vi "PicoScope4000Settings.vi"(0 "handle in":i16, 3 "Unit Info":T1, 5 "error in":errorcluster, 6 "Channel A Settings":T3 {"Coupling" items=["AC", "DC", "IEPE"]; "Bandwidth Limit" items=["Off", "200kHz"]; "Range" items=["10 mV", "20 mV", "50 mV", "100 mV", "200 mV", "500 mV", "1 V", "2 V", "5 V", "10 V", "20 V", "50 V ", "100 V"]}, 7 "Trigger Settings":T4 {"Trigger Direction" items=["Rising", "Falling"]}, 8 "Channel B Settings":T3 {"Coupling" items=["AC", "DC", "IEPE"]; "Bandwidth Limit" items=["Off", "200kHz"]; "Range" items=["10 mV", "20 mV", "50 mV", "100 mV", "200 mV", "500 mV", "1 V", "2 V", "5 V", "10 V", "20 V", "50 V ", "100 V"]}, 10 "Channel C Settings":T2 {"Range" items=["10 mV", "20 mV", "50 mV", "100 mV", "200 mV", "500 mV", "1 V", "2 V", "5 V", "10 V", "20 V", "50 V ", "100 V"]; "Coupling" items=["AC", "DC"]}, 12 "Channel D Settings":T2 {"Range" items=["10 mV", "20 mV", "50 mV", "100 mV", "200 mV", "500 mV", "1 V", "2 V", "5 V", "10 V", "20 V", "50 V ", "100 V"]; "Coupling" items=["AC", "DC"]}, 13 "PicoScope 4262 Ext. Trigger Range":u32(ring) items=["500 mV", "5 V"]) -> (11 "Enabled array":i16[](array[numeric]), 14 "handle out":i16, 19 "error out":errorcluster)   [LabVIEW 2009]
doc: "This VI is used to set up the oscilloscope. The inputs are clusters for setting channel and simple trigger settings. Advanced triggers can be set up using PicoScope4000AdvancedTriggerSettings.vi"
uses:
  ps4000.dll
  PicoScope4000AnalogChannelSettings.ctl
  PicoScope4000AnalogChannelSettingsIEPE.ctl
panel:
  in  "Max ADC value":i16
  # "Note Bandwith Limit not avaiable on all models"
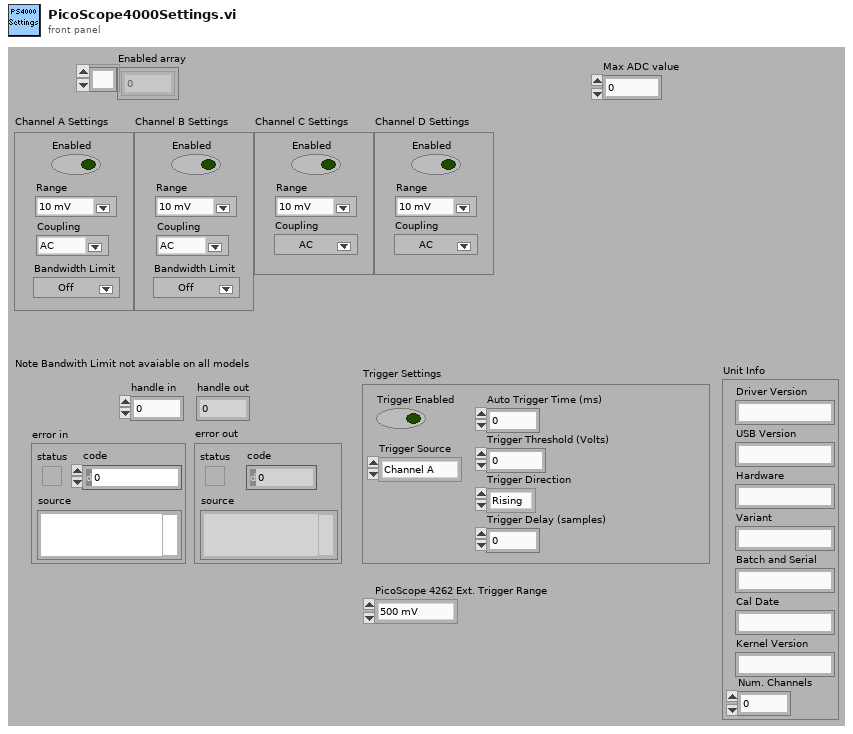
[diagram p1: front panel]
types:
  T1 = cluster{"Driver Version":string, "USB Version":string, "Hardware":string, "Variant":string, "Batch and Serial":string, "Cal Date":string, "Kernel Version":string, "Num. Channels":i16}
  T2 = typedef "PicoScope4000AnalogChannelSettings.ctl" = cluster{"Enabled":bool, "Coupling":i16, "Range":u16}
  T3 = typedef "PicoScope4000AnalogChannelSettingsIEPE.ctl" = cluster{"Enabled":bool, "Range":u16, "Bandwidth Limit":i16, "Coupling":u16}
  T4 = cluster{"Trigger Enabled":bool, "Trigger Source":enum16{"Channel A", "Channel B", "Channel C", "Channel D", "Channel E", "Channel F", "Channel G", "Channel H"}, "Trigger Threshold (Volts)":dbl, "Trigger Direction":u16, "Trigger Delay (samples)":u32, "Auto Trigger Time (ms)":i16}
  T5 = enum16{"Channel A", "Channel B", "Channel C", "Channel D", "Channel E", "Channel F", "Channel G", "Channel H"}
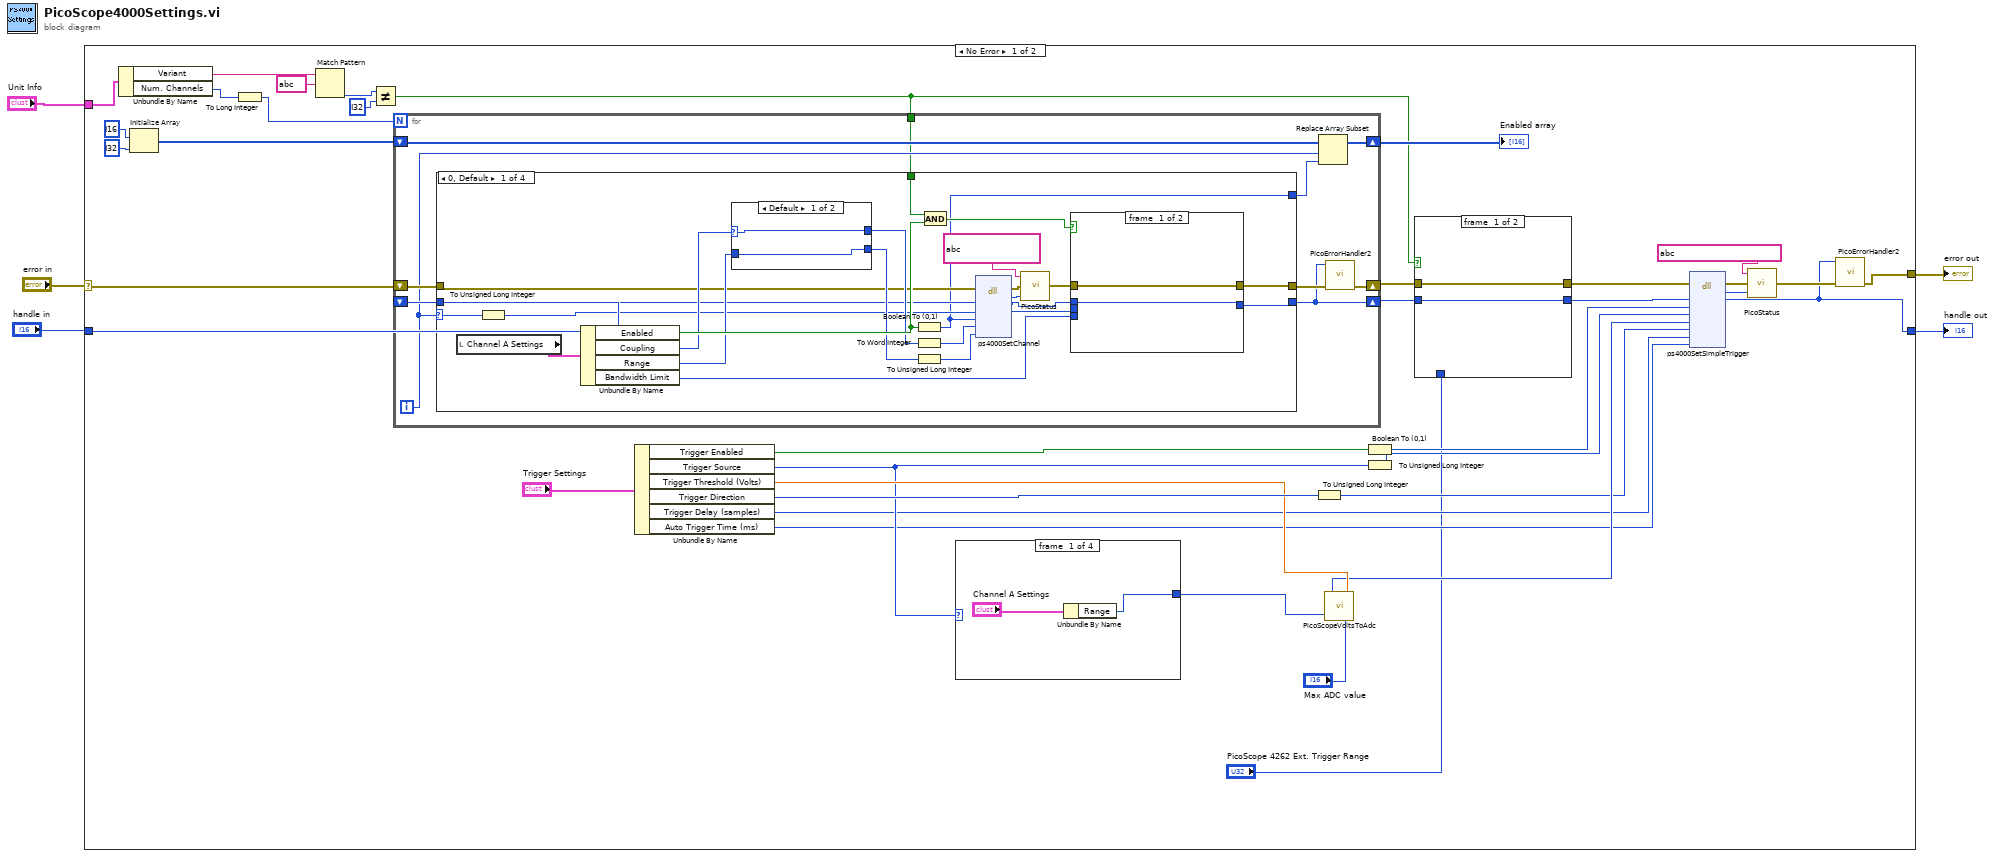
[diagram p0: block diagram]
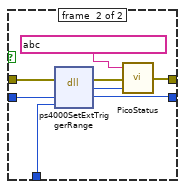
[diagram p2: hidden frame]
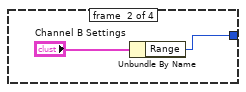
[diagram p3: hidden frame]
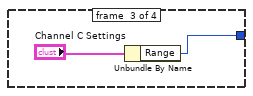
[diagram p4: hidden frame]
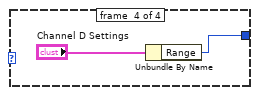
[diagram p5: hidden frame]
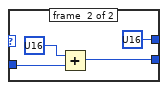
[diagram p6: hidden frame]
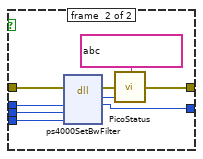
[diagram p7: hidden frame]
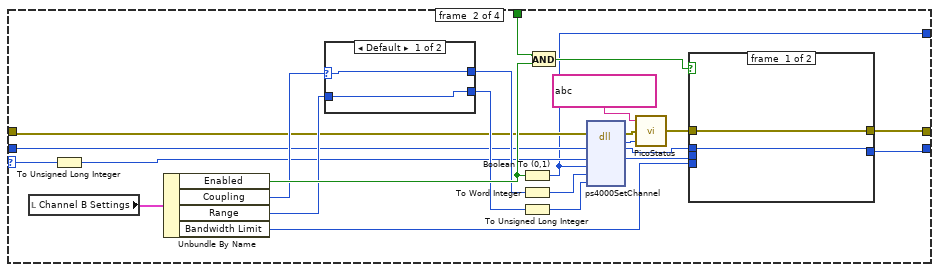
[diagram p8: hidden frame]
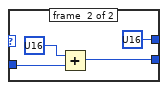
[diagram p9: hidden frame]
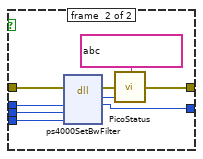
[diagram p10: hidden frame]
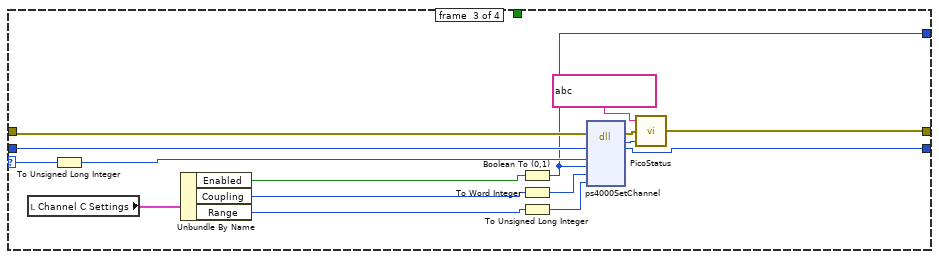
[diagram p11: hidden frame]
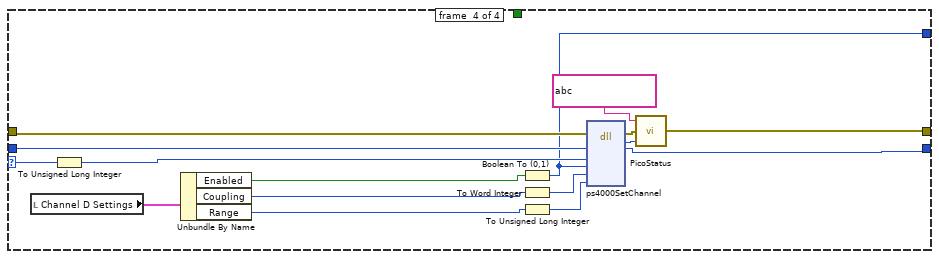
[diagram p12: hidden frame]
diagram:
  n1 = case shown="No Error" "error in" {
    selector: "error in" -> [w39 w187]
    tunnel: "handle in" -> [w40 w186]
    tunnel: [w6 w186] -> w3
    tunnel: [w7 w187] -> w2
    tunnel: "Unit Info" -> [w34 _]
    frame #0 {
      n2 = Unbundle By Name(w34) -> ("Variant"=w27:string, "Num. Channels"=w28:i16)
      n3 = Initialize Array(i16 ? ("element"), i32 ? ("dimension size")) -> (w36:i16[])
      n4 = To Long Integer(number=w28) -> (32bit integer=w33:i32)
      n5 = Match Pattern(string=w27, regular expression=string ?) -> (offset past match=w25:i32)  [unwired: 1 in, 3 out]
      n6 = Not Equal?(x=w25, y=i32 ?) -> (x != y?=w12:bool)
      n7 = for {
        N: w33 -> [_]
        shift-right: [w64] -> w11
        shift-left: w39 -> [w70]
        shift-right: [w63] -> w10
        shift-left: w40 -> [w71]
        shift-right: [w66] -> w35
        shift-left: w36 -> [w67]
        tunnel: w12 -> [w62]
        i -> [w69]
        n8 = case shown="0, Default" w69 {
          selector: w69 -> [w93 w135 w168 w184]
          tunnel: w71 -> [w78 w120 w163 w179]
          tunnel: [w91 w133 w156 w171] -> w65
          tunnel: w70 -> [w79 w121 w164 w180]
          tunnel: [w90 w132 w155 w172] -> w63
          tunnel: [w76 w118 w161 w177] -> w68
          tunnel: w62 -> [w88 w130 _ _]
          frame #0 {
            n9 = local read "Channel A Settings"() -> (w94:T3)
            n10 = To Unsigned Long Integer(number=w93) -> (unsigned 32bit integer=w77:u32)
            n11 = Unbundle By Name(w94) -> ("Enabled"=w87:bool, "Coupling"=w85:u16, "Range"=w82:u16, "Bandwidth Limit"=w86:i16)
            n12 = case shown="Default" w85 {
              selector: w85 -> [w96 _]
              tunnel: w82 -> [w97 w100]
              tunnel: [w97 w101] -> w83
              tunnel: [w96 u16 ? ("Coupling")] -> w84
              frame #0 {
              }
              frame #1 {
                n13 = Add(x=u16 ? ("y"), y=w100) -> (x+y=w101:u16)
              }
            }
            n14 = Boolean To (0,1)(Boolean=w87) -> (0, 1=w76:i16)
            n15 = To Word Integer(number=w84) -> (16bit integer=w75:i16)
            n16 = To Unsigned Long Integer(number=w83) -> (unsigned 32bit integer=w74:u32)
            n17 = And(x=w88, y=w87) -> (x .and. y?=w89:bool)
            n18 = dll-call lib="ps4000.dll" fn="ps4000SetChannel" ("ps3000.dll:_ps3000_open_unit@0")(error in=w79, "handle"=w78, "channel"=w77, "enabled"=w76, "dc"=w75, "range"=w74) -> (error out=w81:errorcluster, "PICO_STATUS"=w80:u32, "handle"=w73:i16, "channel"=w72:u32)  [unwired: 5 in, 1 out]
            n19 = call "PicoStatus.vi"("PICO STATUS"=w80, "error in"=w81, "source"=string ?) -> ("error out"=w92:errorcluster)
            n20 = case shown="True" w89 {
              tunnel: w92 -> [w103 w110]
              tunnel: w73 -> [w102 w109]
              tunnel: [w103 w108] -> w91
              tunnel: [w102 w107] -> w90
              tunnel: w72 -> [_ w105]
              tunnel: w86 -> [_ w104]
              frame #0 {
              }
              frame #1 {
                n21 = dll-call lib="ps4000.dll" fn="ps4000SetBwFilter" ("ps3000.dll:_ps3000_open_unit@0")(error in=w110, "handle"=w109, "channel"=w105, "enable"=w104) -> (error out=w112:errorcluster, "PICO_STATUS"=w106:u32, "handle"=w107:i16)  [unwired: 4 in, 1 out]
                n22 = call "PicoStatus.vi"("PICO STATUS"=w106, "error in"=w112, "source"=string ?) -> ("error out"=w108:errorcluster)
              }
            }
          }
          frame #1 {
            n23 = local read "Channel B Settings"() -> (w113:T3)
            n24 = To Unsigned Long Integer(number=w135) -> (unsigned 32bit integer=w119:u32)
            n25 = Unbundle By Name(w113) -> ("Enabled"=w129:bool, "Coupling"=w127:u16, "Range"=w124:u16, "Bandwidth Limit"=w128:i16)
            n26 = case shown="Default" w127 {
              selector: w127 -> [w137 _]
              tunnel: w124 -> [w138 w141]
              tunnel: [w138 w142] -> w125
              tunnel: [w137 u16 ? ("Coupling")] -> w126
              frame #0 {
              }
              frame #1 {
                n27 = Add(x=u16 ? ("y"), y=w141) -> (x+y=w142:u16)
              }
            }
            n28 = Boolean To (0,1)(Boolean=w129) -> (0, 1=w118:i16)
            n29 = To Word Integer(number=w126) -> (16bit integer=w117:i16)
            n30 = To Unsigned Long Integer(number=w125) -> (unsigned 32bit integer=w116:u32)
            n31 = And(x=w130, y=w129) -> (x .and. y?=w131:bool)
            n32 = dll-call lib="ps4000.dll" fn="ps4000SetChannel" ("ps3000.dll:_ps3000_open_unit@0")(error in=w121, "handle"=w120, "channel"=w119, "enabled"=w118, "dc"=w117, "range"=w116) -> (error out=w123:errorcluster, "PICO_STATUS"=w122:u32, "handle"=w115:i16, "channel"=w114:u32)  [unwired: 5 in, 1 out]
            n33 = call "PicoStatus.vi"("PICO STATUS"=w122, "error in"=w123, "source"=string ?) -> ("error out"=w134:errorcluster)
            n34 = case shown="True" w131 {
              tunnel: w134 -> [w144 w151]
              tunnel: w115 -> [w143 w150]
              tunnel: [w144 w149] -> w133
              tunnel: [w143 w148] -> w132
              tunnel: w114 -> [_ w146]
              tunnel: w128 -> [_ w145]
              frame #0 {
              }
              frame #1 {
                n35 = dll-call lib="ps4000.dll" fn="ps4000SetBwFilter" ("ps3000.dll:_ps3000_open_unit@0")(error in=w151, "handle"=w150, "channel"=w146, "enable"=w145) -> (error out=w153:errorcluster, "PICO_STATUS"=w147:u32, "handle"=w148:i16)  [unwired: 4 in, 1 out]
                n36 = call "PicoStatus.vi"("PICO STATUS"=w147, "error in"=w153, "source"=string ?) -> ("error out"=w149:errorcluster)
              }
            }
          }
          frame #2 {
            n37 = local read "Channel C Settings"() -> (w154:T2)
            n38 = To Unsigned Long Integer(number=w168) -> (unsigned 32bit integer=w162:u32)
            n39 = Unbundle By Name(w154) -> ("Enabled"=w167:bool, "Coupling"=w158:i16, "Range"=w157:u16)
            n40 = Boolean To (0,1)(Boolean=w167) -> (0, 1=w161:i16)
            n41 = To Word Integer(number=w158) -> (16bit integer=w160:i16)
            n42 = To Unsigned Long Integer(number=w157) -> (unsigned 32bit integer=w159:u32)
            n43 = dll-call lib="ps4000.dll" fn="ps4000SetChannel" ("ps3000.dll:_ps3000_open_unit@0")(error in=w164, "handle"=w163, "channel"=w162, "enabled"=w161, "dc"=w160, "range"=w159) -> (error out=w166:errorcluster, "PICO_STATUS"=w165:u32, "handle"=w155:i16)  [unwired: 6 in, 1 out]
            n44 = call "PicoStatus.vi"("PICO STATUS"=w165, "error in"=w166, "source"=string ?) -> ("error out"=w156:errorcluster)
          }
          frame #3 {
            n45 = local read "Channel D Settings"() -> (w170:T2)
            n46 = To Unsigned Long Integer(number=w184) -> (unsigned 32bit integer=w178:u32)
            n47 = Unbundle By Name(w170) -> ("Enabled"=w183:bool, "Coupling"=w174:i16, "Range"=w173:u16)
            n48 = Boolean To (0,1)(Boolean=w183) -> (0, 1=w177:i16)
            n49 = To Word Integer(number=w174) -> (16bit integer=w176:i16)
            n50 = To Unsigned Long Integer(number=w173) -> (unsigned 32bit integer=w175:u32)
            n51 = dll-call lib="ps4000.dll" fn="ps4000SetChannel" ("ps3000.dll:_ps3000_open_unit@0")(error in=w180, "handle"=w179, "channel"=w178, "enabled"=w177, "dc"=w176, "range"=w175) -> (error out=w182:errorcluster, "PICO_STATUS"=w181:u32, "handle"=w172:i16)  [unwired: 6 in, 1 out]
            n52 = call "PicoStatus.vi"("PICO STATUS"=w181, "error in"=w182, "source"=string ?) -> ("error out"=w171:errorcluster)
          }
        }
        n53 = Replace Array Subset(array=w67, new element=w68, index=w69) -> (w66:i16[])
        n54 = call "PicoErrorHandler2.vi"("error in (no error)"=w65, "handle In"=w63) -> ("error out"=w64:errorcluster)  [unwired: 9 in]
      }
      "Enabled array" <- w35
      n55 = Unbundle By Name("Trigger Settings") -> ("Trigger Enabled"=w41:bool, "Trigger Source"=w30:T5, "Trigger Threshold (Volts)"=w31:dbl, "Trigger Direction"=w42:u16, "Trigger Delay (samples)"=w15:u32, "Auto Trigger Time (ms)"=w14:i16)
      n56 = case shown="\"Channel D\"" w30 {
        tunnel: [w54 w56 w58 w60] -> w29
        frame #0 {
          n57 = Unbundle By Name("Channel A Settings") -> ("Range"=w54:u16)
        }
        frame #1 {
          n58 = Unbundle By Name("Channel B Settings") -> ("Range"=w56:u16)
        }
        frame #2 {
          n59 = Unbundle By Name("Channel C Settings") -> ("Range"=w58:u16)
        }
        frame #3 {
          n60 = Unbundle By Name("Channel D Settings") -> ("Range"=w60:u16)
        }
      }
      n61 = To Unsigned Long Integer(number=w42) -> (unsigned 32bit integer=w16:u32)
      n62 = call "PicoScopeVoltsToAdc.vi"("Max_adc"="Max ADC value", "Units"=w31, "Range Index"=w29) -> ("ADC count"=w17:i16)
      n63 = Boolean To (0,1)(Boolean=w41) -> (0, 1=w19:i16)
      n64 = To Unsigned Long Integer(number=w30) -> (unsigned 32bit integer=w18:u32)
      n65 = case shown="True" w12 {
        tunnel: [w45 w49] -> w9
        tunnel: w11 -> [w45 w53]
        tunnel: w10 -> [w44 w52]
        tunnel: [w44 w50] -> w8
        tunnel: "PicoScope 4262 Ext. Trigger Range" -> [_ w51]
        frame #0 {
        }
        frame #1 {
          n66 = dll-call lib="ps4000.dll" fn="ps4000SetExtTriggerRange"(error in=w53, "handle"=w52, "extRange"=w51) -> (error out=w47:errorcluster, "PICO STATUS"=w48:u32, "handle"=w50:i16)  [unwired: 3 in, 1 out]
          n67 = call "PicoStatus.vi"("PICO STATUS"=w48, "error in"=w47, "source"=string ?) -> ("error out"=w49:errorcluster)
        }
      }
      n68 = dll-call lib="ps4000.dll" fn="ps4000SetSimpleTrigger" ("ps3000.dll:_ps3000_open_unit@0")(error in=w9, "handle"=w8, "enabled"=w19, "source"=w18, "threshold"=w17, "direction"=w16, "delay"=w15, "autoTrigger_ms"=w14) -> (error out=w22:errorcluster, "PICO_STATUS"=w23:u32, "handle"=w6:i16)  [unwired: 8 in, 1 out]
      n69 = call "PicoStatus.vi"("PICO STATUS"=w23, "error in"=w22, "source"=string ?) -> ("error out"=w20:errorcluster)
      n70 = call "PicoErrorHandler2.vi"("error in (no error)"=w20, "handle In"=w6) -> ("error out"=w7:errorcluster)  [unwired: 9 in]
    }
    frame #1 {
    }
  }
  "handle out" <- w3
  "error out" <- w2
